vi "toNextDay.vi"(7 "Values":i32[](array[numeric]), 11 "Cron in":T1) -> (3 "Cron out":T1)   [LabVIEW 2013, in "openCron.lvlib" / "Cron.lvclass"]
uses:
  Cron.lvclass
  CronTime -- cluster.ctl
  <vilib>/LabVIEW Open Source Project/Epoch Date & Time/GregorianCal_Month -- enum.ctl
  toNextYear.vi
  <vilib>/LabVIEW Open Source Project/Epoch Date & Time/GregorianCal_MonthLengths.vi
  TimeStamp to Cron Time.vi
  Cron Time to TimeStamp.vi
  <vilib>/LabVIEW Open Source Project/Epoch Date & Time/isLeapYear (integer).vi
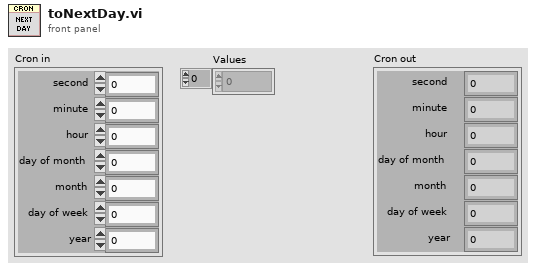
[diagram p1: front panel]
types:
  T1 = typedef "openCron.lvlib/Cron.lvclass/CronTime -- cluster.ctl" = cluster{"second":i32, "minute":i32, "hour":i32, "day of month":i32, "month":i32, "day of week":i32, "year":i32}
  T2 = typedef "GregorianCal_Month -- enum.ctl" = enum16{"January", "February", "March", "April", "May", "June", "July", "August", "September", "October", "November", "December"}
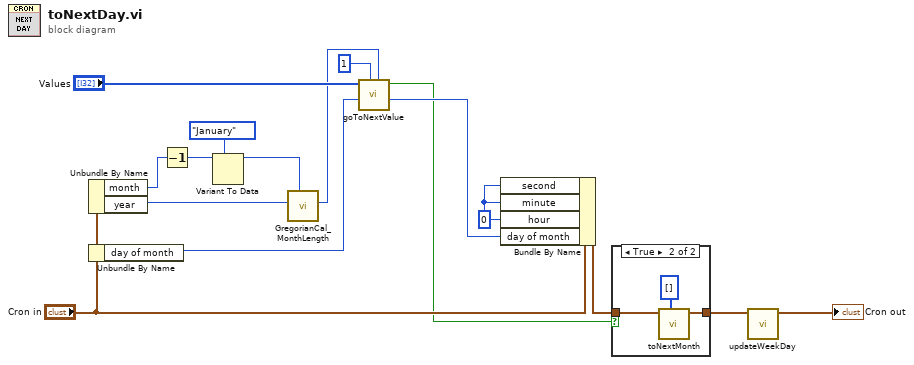
[diagram p0: block diagram]
diagram:
  w16 = 0 ("hour")
  n1 = Unbundle By Name("Cron in") -> ("month"=w12:i32, "year"=w14:i32)
  n2 = Unbundle By Name("Cron in") -> ("day of month"=w3:i32)
  n3 = Decrement(x=w12) -> (x-1=w9:i32)
  n4 = Variant To Data(type=GregorianCal_Month_--_enum."January" ("Month"), Variant=w9) -> (data=w10:T2)  [unwired: 1 in, 1 out]
  n5 = call <vilib>:"GregorianCal_MonthLength.vi"("Month"=w10, "Year (0: this year)"=w14) -> ("Nb Days"=w5:i32)  [unwired: 9 in]
  n6 = call "goToNextValue.vi"("maxValue"=w5, "min Value"=1 ("lower limit"), "value in"=w3, "Values Pool"="Values") -> ("next value"=w2:i32, "RolledOver"=w1:bool)  [unwired: 6 in]
  n7 = Bundle By Name(cluster="Cron in", "second"=w16, "minute"=w16, "hour"=w16, "day of month"=w2) -> (w15:T1)
  n8 = case shown="True" w1 {
    tunnel: w15 -> [w17 w20]
    tunnel: [w17 w19] -> w7
    frame False {
    }
    frame True {
      n9 = call "toNextMonth.vi"("Values"=i32[] [], "Cron in"=w20) -> ("Cron out"=w19:T1)  [unwired: 9 in]
    }
  }
  n10 = call "updateWeekDay.vi"("Cron in"=w7) -> ("Cron Time"=→"Cron out":T1)  [unwired: 10 in]
